vi "WaitOnTestComplete.vi"(8 "error in (no error)":errorcluster, 11 "TestCase in":refnum<class "TestCase.lvclass">) -> (0 "error out":errorcluster, 3 "TestCase out":refnum<class "TestCase.lvclass">)   [LabVIEW 2013, in "TestCase.lvclass"]
doc: "Insert WaitOnTestComplete at the end of setUp test hook if the test hook VI opens any references that are needed by the test methods at run time."
uses:
  TestCase.lvclass
  TestCase.lvclass/TestCase.ctl
panel:
  # "JKI VI Tester for LabVIEW\nhttp://jkisoft.com/vi-tester\nCopyright (C) 2007-2009, JKI <info@jkisoft.com>\nALL RIGHTS RESERVED"
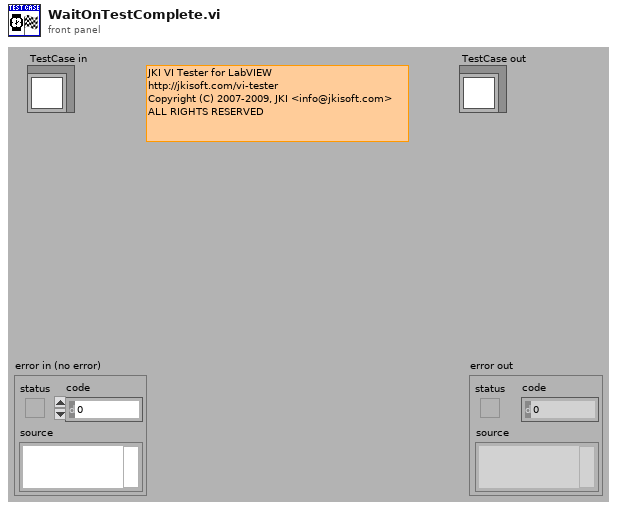
[diagram p1: front panel]
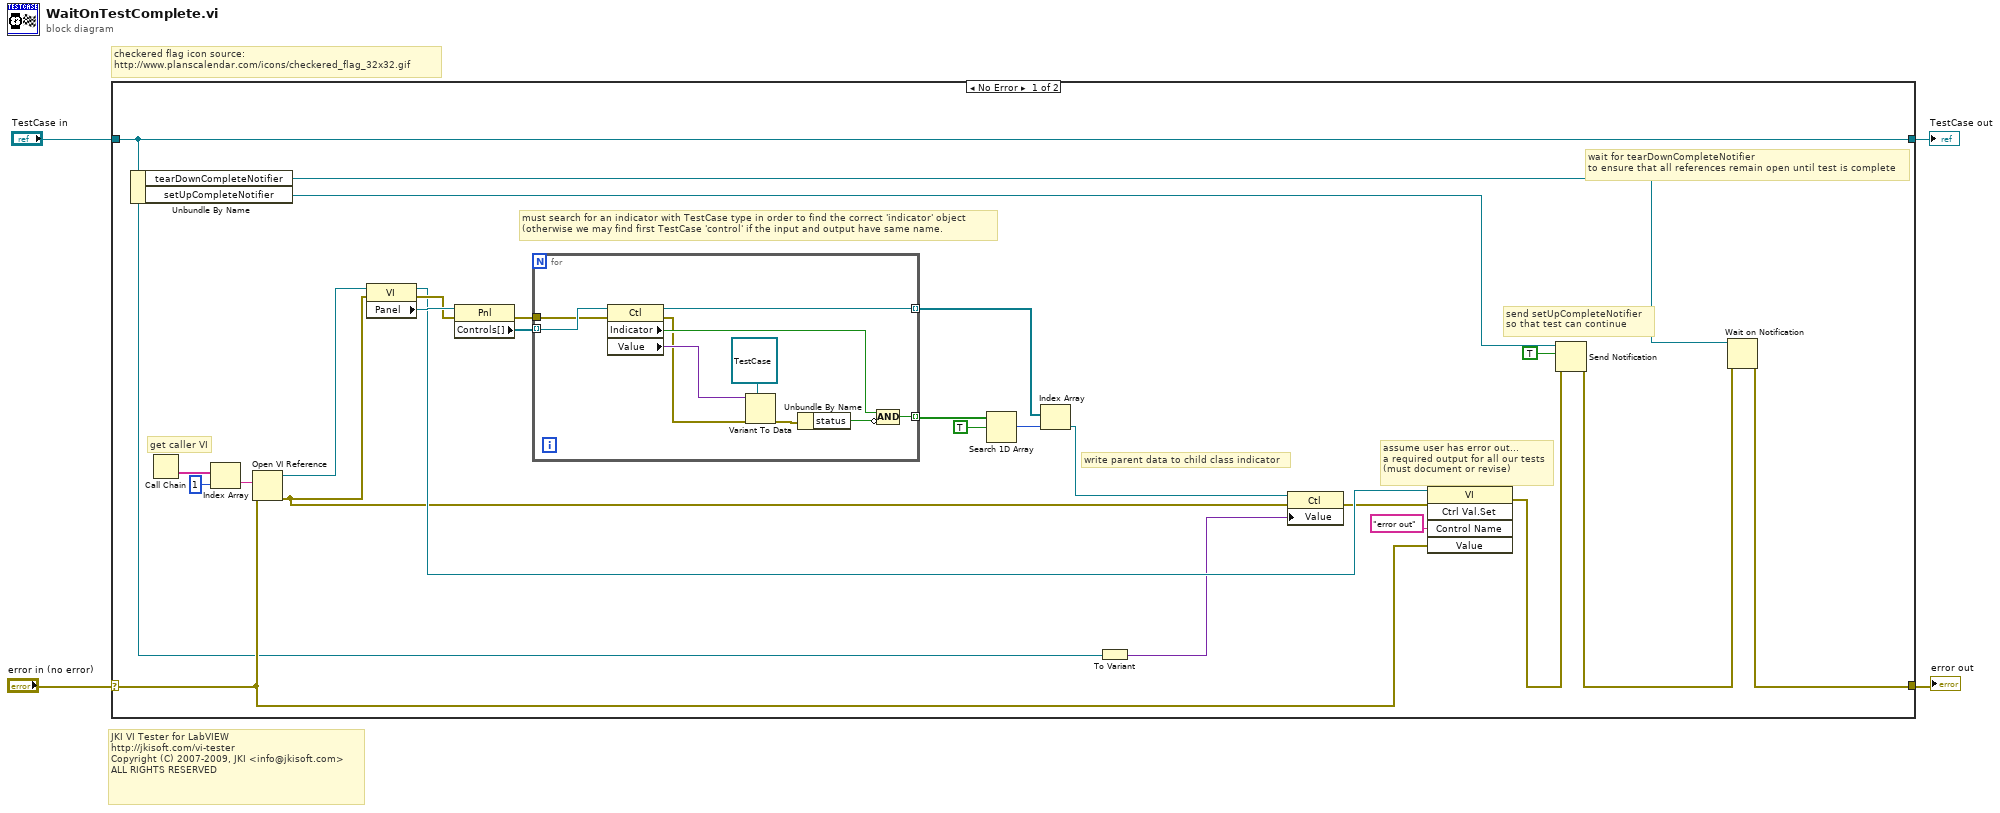
[diagram p0: block diagram]
diagram:
  # "JKI VI Tester for LabVIEW\nhttp://jkisoft.com/vi-tester\nCopyright (C) 2007-2009, JKI <info@jkisoft.com>\nALL RIGHTS RESERVED"
  # "checkered flag icon source:\nhttp://www.planscalendar.com/icons/checkered_flag_32x32.gif"
  n1 = case shown="No Error" "error in (no error)" {
    selector: "error in (no error)" -> [w11 w42]
    tunnel: [w29 w42] -> w3
    tunnel: [w8 w41] -> w1
    tunnel: "TestCase in" -> [w8 w41]
    frame No Error {
      # "write parent data to child class indicator"
      # "get caller VI"
      # "must search for an indicator with TestCase type in order to find the correct 'indicator' object\n(otherwise we may find first TestCase 'control' if the input and output have same name."
      # "assume user has error out...\na required output for all our tests\n(must document or revise)"
      # "wait for tearDownCompleteNotifier\nto ensure that all references remain open until test is complete"
      # "send setUpCompleteNotifier\nso that test can continue"
      n2 = Unbundle By Name(w8) -> ("tearDownCompleteNotifier"=w30:refnum<notifier>, "setUpCompleteNotifier"=w28:refnum<notifier>)
      n3 = Call Chain() -> (call chain=w25:string[])
      n4 = Index Array(array=w25, index=1) -> (element=w23:string)
      n5 = Open VI Reference(vi path=w23, error in (no error)=w11) -> (vi reference=w10:refnum<vi>, error out=w9:errorcluster)  [unwired: 4 in]
      n6 = property class="VI"(reference=w10, error in=w9) -> (reference out=w13:refnum<vi>, error out=w20:errorcluster, "Panel"=w22:refnum<vi>)
      n7 = property class="Pnl"(reference=w22, error in=w20) -> (error out=w19:errorcluster, "Controls[]"=w21:refnum<vi>[])  [unwired: 1 out]
      n8 = for {
        tunnel: w21 -> [w40] mode=indexing
        tunnel: [w34] -> w18 mode=indexing
        tunnel: w19 -> [w32]
        tunnel: [w31] -> w15 mode=indexing
        n9 = property class="Ctl"(reference=w40, error in=w32) -> (reference out=w31:refnum<vi>, error out=w33:errorcluster, "Indicator"=w35:bool, "Value"=w38:variant)
        n10 = Variant To Data(error in=w33, type=refnum<class "TestCase.lvclass"> refnum ("TestCase.lvclass"), Variant=w38) -> (error out=w37:errorcluster)  [unwired: 1 out]
        n11 = Unbundle By Name(w37) -> ("status"=w36:bool)
        n12 = Compound Arithmetic op=AND(w35, invert w36) -> (w34:bool)
      }
      n13 = Search 1D Array(1D array=w18, element=TRUE) -> (index of element=w16:i32)  [unwired: 1 in]
      n14 = Index Array(array=w15, index=w16) -> (element=w6:refnum<vi>)
      n15 = To Variant(anything=w8) -> (Variant=w5:variant)
      n16 = property class="Ctl"(reference=w6, error in=w9, "Value"=w5) -> (error out=w7:errorcluster)  [unwired: 1 out]
      n17 = invoke class="VI" method="Ctrl Val.Set"(reference=w13, error in=w7, "Control Name"="error out", "Value"=w11) -> (error out=w12:errorcluster)  [unwired: 1 in, 4 out]
      n18 = Send Notification(notification=TRUE, notifier=w28, error in (no error)=w12) -> (error out=w27:errorcluster)  [unwired: 1 out]
      n19 = Wait on Notification(notifier=w30, error in (no error)=w27) -> (error out=w29:errorcluster)  [unwired: 2 in, 3 out]
    }
    frame Error {
    }
  }
  "error out" <- w3
  "TestCase out" <- w1
